vi "Init Msg Default.vi"() -> (3 "Stop Msg out":refnum<class "Stop Msg.lvclass">)   [LabVIEW 2020, in "jettl.lvlib" / "Stop jettl Msg.lvlib" / "Stop Msg.lvlib" / "Stop Msg.lvclass"]
uses:
  Stop Msg.lvclass
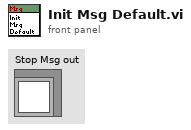
[diagram p1: front panel]
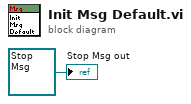
[diagram p0: block diagram]
diagram:
  "Stop Msg out" <- refnum<class "Stop Msg.lvclass"> refnum ("Destroy Msg in")
